vi "update tree column header.vi"(7 "Interpret as Unicode (T)":bool=TRUE, 8 "error in (no error)":errorcluster, 10 "Column Header":string[](array[string]), 11 "Tree Refnum in":refnum<vi>) -> (0 "error out":errorcluster, 3 "Tree Refnum out":refnum<vi>)   [LabVIEW 2019, in "Language Selection.lvlib"]
doc: "- - -\nCopyright (c) 2026, Merecs Engineering GmbH"
uses:
  Language Selection.lvlib
panel:
  # "Connector Pane"
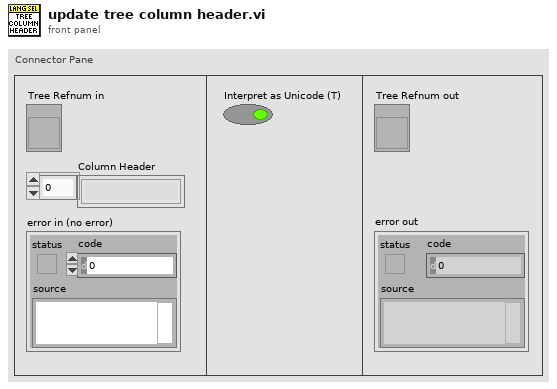
[diagram p1: front panel]
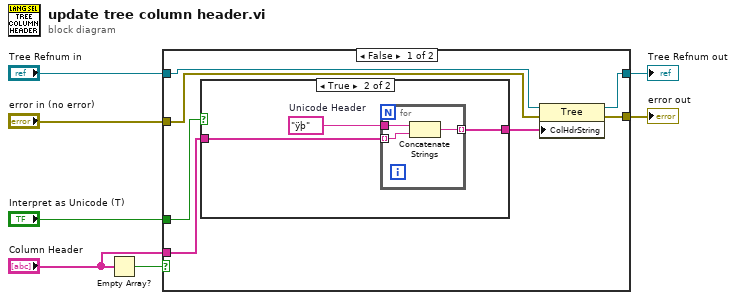
[diagram p0: block diagram]
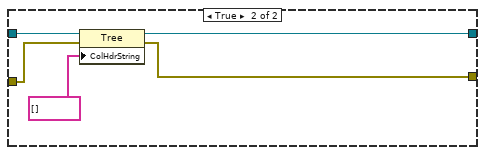
[diagram p3: hidden frame]
diagram:
  n1 = Empty Array?(array="Column Header") -> (empty?=w1:bool)
  n2 = case shown="False" w1 {
    tunnel: "Column Header" -> [w14 _]
    tunnel: [w13 w25] -> w5
    tunnel: "error in (no error)" -> [w12 w24]
    tunnel: "Tree Refnum in" -> [w11 w23]
    tunnel: "Interpret as Unicode (T)" -> [w10 _]
    tunnel: [w9 w26] -> w6
    frame False {
      n3 = case shown="True" w10 {
        tunnel: w14 -> [w15 w18]
        tunnel: [w15 w17] -> w8
        frame False {
        }
        frame True {
          w16 = "ÿþ"  # Unicode Header
          n4 = for {
            tunnel: w18 -> [w21] mode=indexing
            tunnel: [w20] -> w17 mode=indexing
            tunnel: w16 -> [w19]
            n5 = Concatenate Strings(w19, w21) -> (w20:string)
          }
        }
      }
      n6 = property class="Tree"(reference=w11, error in=w12, "ColHdrString"=w8) -> (reference out=w9:refnum<vi>, error out=w13:errorcluster)
    }
    frame True {
      n7 = property class="Tree"(reference=w23, error in=w24, "ColHdrString"=string[] []) -> (reference out=w26:refnum<vi>, error out=w25:errorcluster)
    }
  }
  "error out" <- w5
  "Tree Refnum out" <- w6
